vi "Config_File_Read_Block.vi"(8 "error in (no error)":errorcluster={"status"=FALSE, "code"=0, "source"="\"\""}, 11 "Local package path":string) -> (0 "error out":errorcluster={"status"=FALSE, "code"=0, "source"="\"\""}, 2 "status ok":bool, 3 "Raw bytes":string)   [LabVIEW 2026]
doc: "INTENT: Read locally stored package. LOGIC: Check path, read complete content, check size limits before decoding."
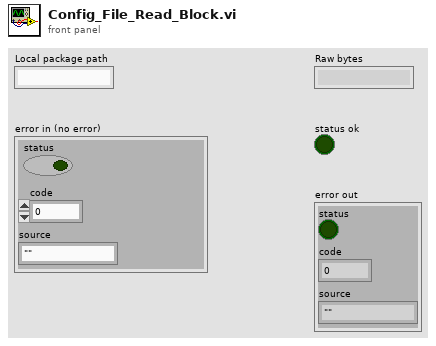
[diagram p1: front panel]
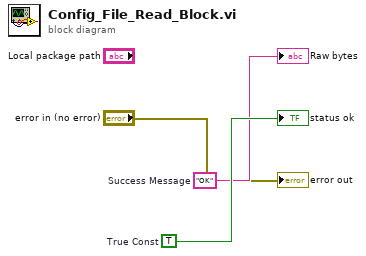
[diagram p0: block diagram]
diagram:
  w3 = TRUE  # True Const
  w2 = "OK"  # Success Message
  "Raw bytes" <- w2
  "status ok" <- w3
  "error out" <- "error in (no error)"
